vi "PhotonMultiTargetPNPResult_pack.vi"(9 "MultiTargetPNP_Result":T1={"PhotonPNPResult"={"IsPresent"=FALSE, "bestReprojErr"=0.0, "altReprojErr"=0.0, "ambiguity"=0.0, "Best"={"TRANSLATION3D"={"X"=0.0, "Y"=0.0, "Z"=0.0}, "ROTATION3D"={"Q_quaternion"={"R"=1.0, "V"=[0.0, 0.0, 0.0]}}, "XF"=FALSE}, "Alt"={"TRANSLATION3D"={"X"=0.0, "Y"=0.0, "Z"=0.0}, "ROTATION3D"={"Q_quaternion"={"R"=1.0, "V"=[0.0, 0.0, 0.0]}}, "XF"=FALSE}}, "FiducialIDsUsed"=[]} {"PhotonPNPResult"."Alt"."TRANSLATION3D"."Z" format="%14.3f"; "PhotonPNPResult"."Alt"."TRANSLATION3D"."Y" format="%14.3f"; "PhotonPNPResult"."Alt"."TRANSLATION3D"."X" format="%14.3f"; "PhotonPNPResult"."Best"."TRANSLATION3D"."Z" format="%14.3f"; "PhotonPNPResult"."Best"."TRANSLATION3D"."Y" format="%14.3f"; "PhotonPNPResult"."Best"."TRANSLATION3D"."X" format="%14.3f"}, 11 "RawData In":u8[](array[numeric])) -> (3 "RawData Out":u8[](array[numeric]))   [LabVIEW 2019, in "PhotonVisionLib.lvlib"]
doc: "Encode a MultiTargetPNPResult cluster into an array of bytes.\n\nInputs:\n - MultiTagetPNPResult -- cluster containing the data to pack.\n\nOutputs:\n - RawDataOut -- Byte array containing the encoded data."
uses:
  PhotonVisionLib.lvlib
  TypeDef/PhotonMultiTargetPNPResultType.ctl
  TypeDef/PhotonPNPResultType.ctl
  <vilib>/Rock Robotics/WPI/ThirdParty/JAS_Junk/TrajLib/TypeDef/TRANSFORM3D.ctl
  <vilib>/Rock Robotics/WPI/ThirdParty/JAS_Junk/TrajLib/TypeDef/TRANSLATION3D.ctl
  <vilib>/Rock Robotics/WPI/ThirdParty/JAS_Junk/TrajLib/TypeDef/ROTATION3D.ctl
  <vilib>/Rock Robotics/WPI/ThirdParty/JAS_Junk/TrajLib/TypeDef/QUATERNION.ctl
  Packet_encode_Transform3d.vi
  Packet_encode_FLT64.vi
  <vilib>/Rock Robotics/WPI/ThirdParty/JAS_Junk/TrajLib/VI/Transform3d_GetXYZ.vi
  <vilib>/Rock Robotics/WPI/ThirdParty/JAS_Junk/TrajLib/VI/Transform3d_GetRotation3d.vi
  <vilib>/Rock Robotics/WPI/ThirdParty/JAS_Junk/TrajLib/VI/Rotation3d_GetQuaterion.vi
  <vilib>/Rock Robotics/WPI/ThirdParty/JAS_Junk/TrajLib/VI/Quaternion_Get_All.vi
  <vilib>/Rock Robotics/WPI/ThirdParty/JAS_Junk/TrajLib/VI/Transform3d_GetTranslation3d.vi
  <vilib>/Rock Robotics/WPI/ThirdParty/JAS_Junk/TrajLib/VI/Translation3d_GetXYZ.vi
  <vilib>/Rock Robotics/WPI/ThirdParty/JAS_Junk/TrajLib/Trajectory_Library.lvlib
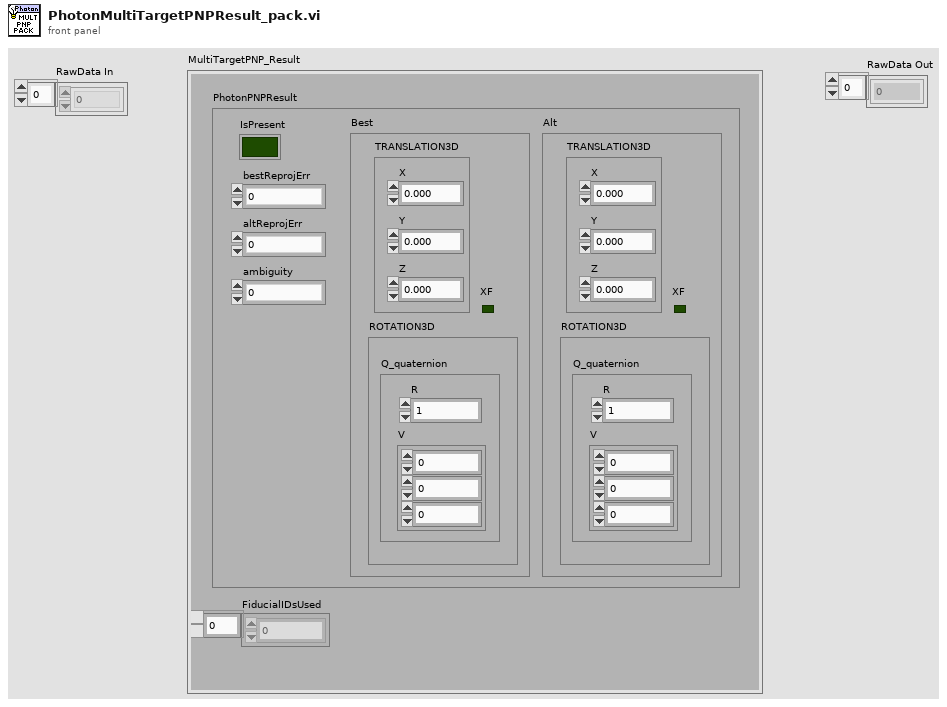
[diagram p1: front panel]
types:
  T1 = typedef "PhotonVisionLib.lvlib/PhotonMultiTargetPNPResultType.ctl" = cluster{"PhotonPNPResult":T2, "FiducialIDsUsed":i16[]}
  T2 = typedef "PhotonVisionLib.lvlib/PhotonPNPResultType.ctl" = cluster{"IsPresent":bool, "bestReprojErr":dbl, "altReprojErr":dbl, "ambiguity":dbl, "Best":T3, "Alt":T3}
  T3 = typedef "Trajectory_Library.lvlib/TRANSFORM3D.ctl" = cluster{"TRANSLATION3D":T4, "ROTATION3D":T5, "XF":bool}
  T4 = typedef "Trajectory_Library.lvlib/TRANSLATION3D.ctl" = cluster{"X":dbl, "Y":dbl, "Z":dbl}
  T5 = typedef "Trajectory_Library.lvlib/ROTATION3D.ctl" = cluster{"Q_quaternion":T6}
  T6 = typedef "Trajectory_Library.lvlib/QUATERNION.ctl" = cluster{"R":dbl, "V":dbl[]}
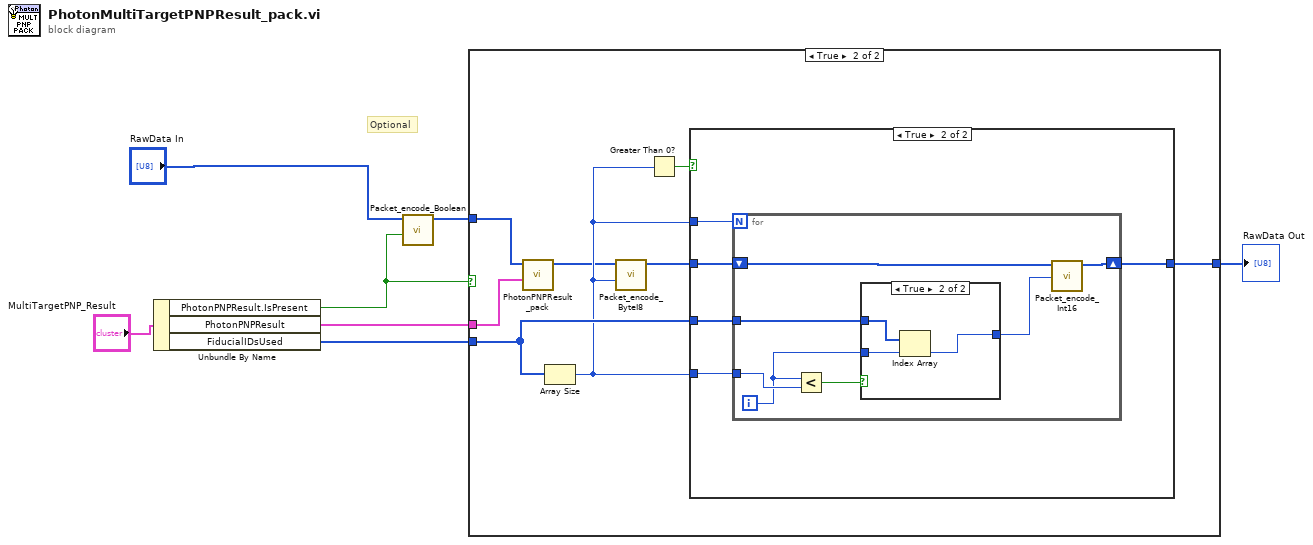
[diagram p0: block diagram]
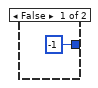
[diagram p4: hidden frame]
diagram:
  # "Optional"
  n1 = Unbundle By Name("MultiTargetPNP_Result") -> ("PhotonPNPResult.IsPresent"=w2:bool, "PhotonPNPResult"=w5:T2, "FiducialIDsUsed"=w6:i16[])
  n2 = call "Packet_encode_Boolean.vi"("Boolean_Value"=w2, "RawData In"="RawData In") -> ("RawData Out"=w3:u8[])  [unwired: 9 in]
  n3 = case shown="True" w2 {
    tunnel: w6 -> [_ w16]
    tunnel: w5 -> [_ w11]
    tunnel: [w8 w10] -> w4
    tunnel: w3 -> [w8 w9]
    frame False {
    }
    frame True {
      n4 = call "PhotonPNPResult_pack.vi"("PNP_Result"=w11, "RawData In"=w9) -> ("RawData Out"=w12:u8[])  [unwired: 9 in]
      n5 = Array Size(array=w16) -> (size(s)=w13:i32)
      n6 = call "Packet_encode_ByteI8.vi"("Int8_Value"=w13, "RawData In"=w12) -> ("RawData Out"=w15:u8[])  [unwired: 9 in]
      n7 = Greater Than 0?(x=w13) -> (x > 0?=w14:bool)
      n8 = case shown="True" w14 {
        tunnel: w16 -> [_ w22]
        tunnel: [w17 w21] -> w10
        tunnel: w15 -> [w17 w20]
        tunnel: w13 -> [_ w19]
        tunnel: w13 -> [_ w18]
        frame False {
        }
        frame True {
          n9 = for {
            N: w18 -> [_]
            tunnel: w22 -> [w26]
            shift-right: [w23] -> w21
            shift-left: w20 -> [w29]
            tunnel: w19 -> [w28]
            i -> [w25]
            n10 = Less?(x=w25, y=w28) -> (x < y?=w27:bool)
            n11 = case shown="True" w27 {
              tunnel: w26 -> [_ w33]
              tunnel: w25 -> [_ w32]
              tunnel: [i16 -1 ("FiducialIDsUsed") w31] -> w24
              frame False {
              }
              frame True {
                n12 = Index Array(array=w33, index=w32) -> (element=w31:i16)
              }
            }
            n13 = call "Packet_encode_Int16.vi"("Int16_Value"=w24, "RawData In"=w29) -> ("RawData Out"=w23:u8[])  [unwired: 9 in]
          }
        }
      }
    }
  }
  "RawData Out" <- w4
